vi "delete module from engine.vi"(8 "error in":errorcluster, 10 "module ID":string, 11 "engine configuration in":refnum<class "engine configuration.lvclass">) -> (0 "error out":errorcluster, 3 "engine configuration out":refnum<class "engine configuration.lvclass">)   [LabVIEW 2014, in "engine configuration.lvclass"]
doc: "Unregisters a module and deletes all of its configured mappings from the engine configuration."
uses:
  engine configuration.lvclass
  engine configuration.lvclass/engine configuration.ctl
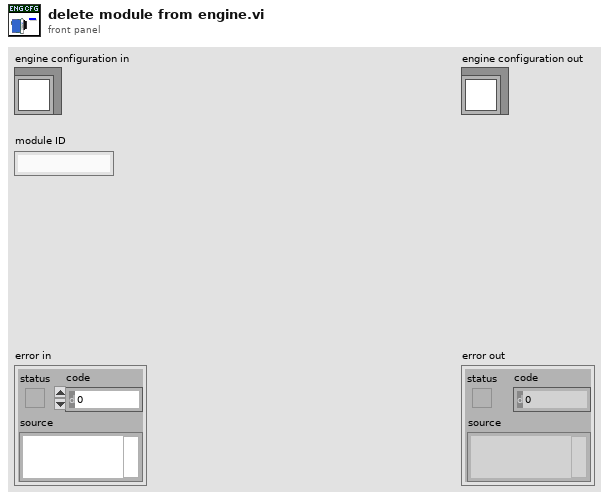
[diagram p1: front panel]
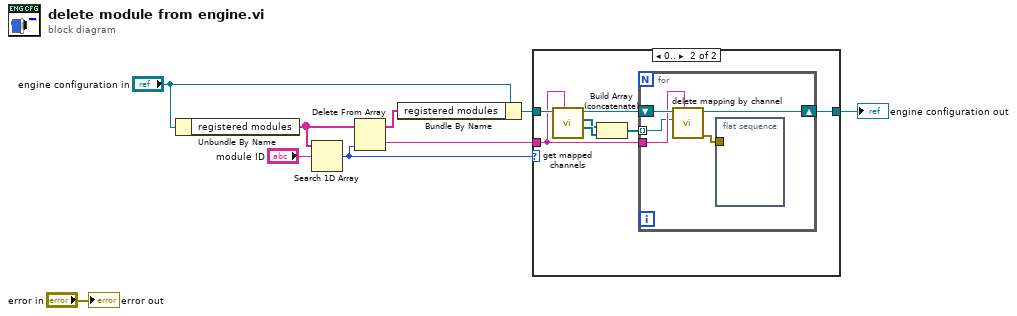
[diagram p0: block diagram]
diagram:
  n1 = Unbundle By Name("engine configuration in") -> ("registered modules"=w4:string[])
  n2 = Search 1D Array(1D array=w4, element="module ID") -> (index of element=w3:i32)  [unwired: 1 in]
  n3 = Delete From Array(array=w4, index=w3) -> (deleted portion=w2:string, array with subset deleted=w1:string[])  [unwired: 1 in]
  n4 = Bundle By Name(cluster="engine configuration in", "registered modules"=w1) -> (w5:refnum<class "engine configuration.lvclass">)
  n5 = case shown="0.." w3 {
    tunnel: w5 -> [w10 w17]
    tunnel: [w10 w12] -> w6
    tunnel: w2 -> [_ w11]
    frame ..-1 {
    }
    frame 0.. {
      n6 = call-dynamic "get mapped channels.vi"("owner"=w11, "engine configuration in"=w17) -> ("write channels"=w16:refnum<class "TBM channel.lvclass">[], "read channels"=w15:refnum<class "TBM channel.lvclass">[], "engine configuration out"=w13:refnum<class "engine configuration.lvclass">)  [unwired: 5 in, 2 out]
      n7 = Build Array (concatenate)(w15, w16) -> (w14:refnum<class "TBM channel.lvclass">[])
      n8 = for {
        tunnel: w14 -> [w20] mode=indexing
        shift-right: [w19] -> w12
        shift-left: w13 -> [w22]
        tunnel: w11 -> [w21]
        n9 = call "delete mapping by channel.vi"("owner ID"=w21, "channel"=w20, "engine configuration in"=w22) -> ("error out"=w18:errorcluster, "engine configuration out"=w19:refnum<class "engine configuration.lvclass">)  [unwired: 7 in]
        n10 = flat-sequence {
          tunnel: w18 -> [_]
          frame #0 {
          }
        }
      }
    }
  }
  "engine configuration out" <- w6
  "error out" <- "error in"
